vi "Wrap proxy config.vi"(6 "PROXY CONFIGURATION":T1[](array[typedef])=[{"PROTOCOL"="tcp", "DIRECTION"="outbound", "LISTEN ADRESS"="", "LISTEN PORT"=61000, "FWR DST ADRESS"="", "FWR DST PORT"=0, "FWR SRC ADRESS"="", "FWR SRC PORT"=0}, {"PROTOCOL"="tcp", "DIRECTION"="outbound", "LISTEN ADRESS"="", "LISTEN PORT"=61001, "FWR DST ADRESS"="", "FWR DST PORT"=0, "FWR SRC ADRESS"="", "FWR SRC PORT"=0}, {"PROTOCOL"="udp", "DIRECTION"="outbound", "LISTEN ADRESS"="", "LISTEN PORT"=61001, "FWR DST ADRESS"="", "FWR DST PORT"=0, "FWR SRC ADRESS"="", "FWR SRC PORT"=0}, {"PROTOCOL"="udp", "DIRECTION"="inbound", "LISTEN ADRESS"="", "LISTEN PORT"=62001, "FWR DST ADRESS"="", "FWR DST PORT"=0, "FWR SRC ADRESS"="", "FWR SRC PORT"=0}], 7 "PORT CONFIGURATION":T3(array[cluster])=[{"Name"="ENET1", "IPv4 Address"="192.168.1.3", "IPv4 Subnet Mask"="255.255.255.0", "IPv6 Address"="", "is tagged?"=FALSE, "VLAN ID"=0}], 8 "error in":errorcluster, 10 "DUT Info":T2={"DUT IP"="192.168.1.12", "DUT Username"="Administrator", "DUT Password"="NITEST", "DUT SSH PORT"=22, "DUT FWD TEST PORT"=62000, "DUT MAC ADDRESS"="02:00:08:38:2d:37"}, 11 "XNET INTERFACE":string="ENET1") -> (0 "error out":errorcluster, 3 "config":string)   [LabVIEW 2026]
uses:
  DUT Info.ctl
  Proxy Config.ctl
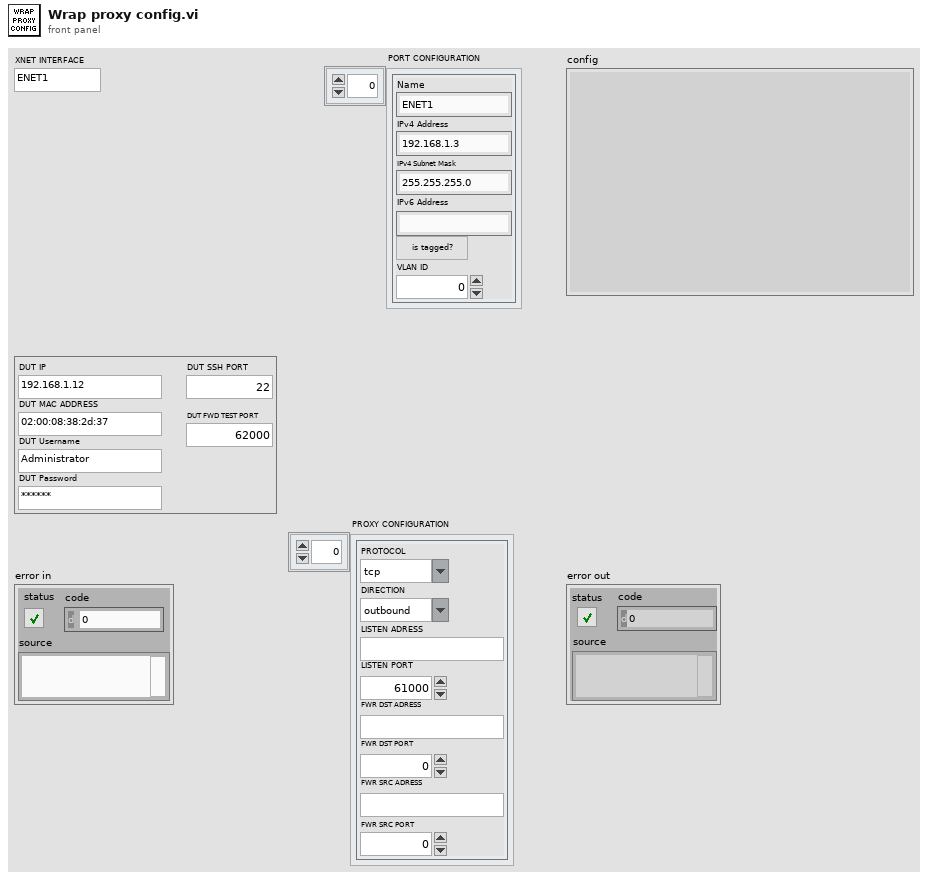
[diagram p1: front panel]
types:
  T1 = typedef "Proxy Config.ctl" = cluster{"PROTOCOL":string, "DIRECTION":string, "LISTEN ADRESS":string, "LISTEN PORT":u16, "FWR DST ADRESS":string, "FWR DST PORT":u16, "FWR SRC ADRESS":string, "FWR SRC PORT":u16}
  T2 = typedef "DUT Info.ctl" = cluster{"DUT IP":string, "DUT Username":string, "DUT Password":string, "DUT SSH PORT":u16, "DUT FWD TEST PORT":u16, "DUT MAC ADDRESS":string}
  T3 = cluster{"Name":string, "IPv4 Address":string, "IPv4 Subnet Mask":string, "IPv6 Address":string, "is tagged?":bool, "VLAN ID":u16}[]
  T4 = cluster{"Name":string, "IPv4 Address":string, "IPv4 Subnet Mask":string, "IPv6 Address":string, "is tagged?":bool, "VLAN ID":u16}
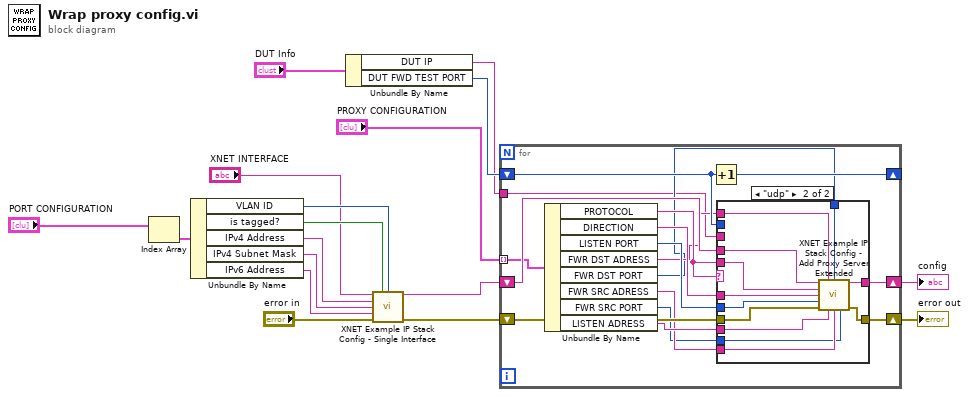
[diagram p0: block diagram]
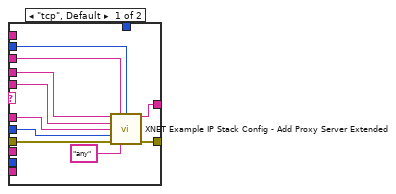
[diagram p2: hidden frame]
diagram:
  n1 = Index Array(array="PORT CONFIGURATION") -> (element=w17:T4)  [unwired: 1 in]
  n2 = Unbundle By Name(w17) -> ("VLAN ID"=w12:u16, "is tagged?"=w13:bool, "IPv4 Address"=w16:string, "IPv4 Subnet Mask"=w15:string, "IPv6 Address"=w14:string)
  n3 = Unbundle By Name("DUT Info") -> ("DUT IP"=w9:string, "DUT FWD TEST PORT"=w10:u16)
  n4 = call <vilib>:"XNET Example IP Stack Config - Single Interface.vi"("XNET interface"="XNET INTERFACE", "is tagged?"=w13, "VLAN ID"=w12, "IPv4 address"=w16, "IPv4 subnet mask"=w15, "IPv6 address"=w14, "error in (no error)"="error in") -> ("config"=w11:string, "error out"=w3:errorcluster)  [unwired: 7 in]
  n5 = for {
    tunnel: w9 -> [w18]
    shift-right: [w32] -> w8
    shift-left: w11 -> [w33]
    tunnel: "PROXY CONFIGURATION" -> [w31] mode=indexing
    shift-right: [w27] -> _
    shift-left: w10 -> [w28]
    shift-right: [w26] -> w1
    shift-left: w3 -> [w25]
    n6 = Unbundle By Name(w31) -> ("PROTOCOL"=w24:string, "DIRECTION"=w30:string, "LISTEN PORT"=w29:u16, "FWR DST ADRESS"=w20:string, "FWR DST PORT"=w19:u16, "FWR SRC ADRESS"=w22:string, "FWR SRC PORT"=w21:u16, "LISTEN ADRESS"=w23:string)
    n7 = Increment(x=w28) -> (x+1=w27:u16)
    n8 = case shown="\"udp\"" w24 {
      tunnel: w33 -> [w43 w44]
      tunnel: w18 -> [w42 _]
      tunnel: [w41 w55] -> w32
      tunnel: w30 -> [w40 w54]
      tunnel: w29 -> [w39 w53]
      tunnel: w28 -> [w38 _]
      tunnel: [w37 w52] -> w26
      tunnel: w25 -> [w36 w51]
      tunnel: w24 -> [w35 w50]
      tunnel: w23 -> [_ w49]
      tunnel: w22 -> [_ w48]
      tunnel: w21 -> [_ w47]
      tunnel: w20 -> [_ w46]
      tunnel: w19 -> [_ w45]
      frame "tcp", Default {
        n9 = call "XNET Example IP Stack Config - Add Proxy Server Extended.vi"("config in"=w43, "forwarding destination address"=w42, "forwarding destination port"=w38, "protocol"=w35, "direction"=w40, "listen port"=w39, "error in (no error)"=w36, "listen address"="any") -> ("config out"=w41:string, "error out"=w37:errorcluster)  [unwired: 6 in]
      }
      frame "udp" {
        n10 = call "XNET Example IP Stack Config - Add Proxy Server Extended.vi"("config in"=w44, "forwarding destination address"=w46, "forwarding destination port"=w45, "protocol"=w50, "direction"=w54, "listen port"=w53, "error in (no error)"=w51, "listen address"=w49, "forwarding source address"=w48, "forwarding source port"=w47) -> ("config out"=w55:string, "error out"=w52:errorcluster)  [unwired: 4 in]
      }
    }
  }
  "config" <- w8
  "error out" <- w1
